vi "GetHSL.vi"(0 "ColorHLS in":refnum<class "ColorHSL.lvclass">, 11 "error in (no error)":errorcluster) -> (4 "ColorHLS out":refnum<class "ColorHSL.lvclass">, 6 "H (°)":dbl, 8 "S (%)":dbl, 10 "L (%)":dbl, 15 "error out":errorcluster)   [LabVIEW 2021, in "Picture2D.lvlib" / "ColorHSL.lvclass"]
uses:
  ColorHSL.lvclass
  ColorHSL.lvclass/ColorHSL.ctl
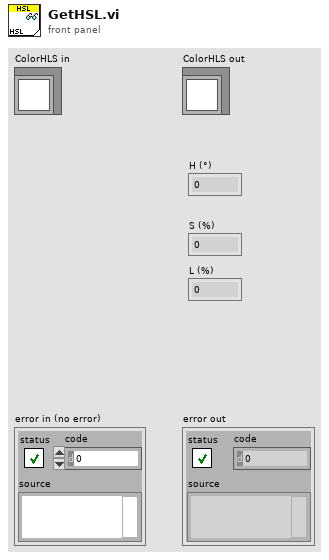
[diagram p1: front panel]
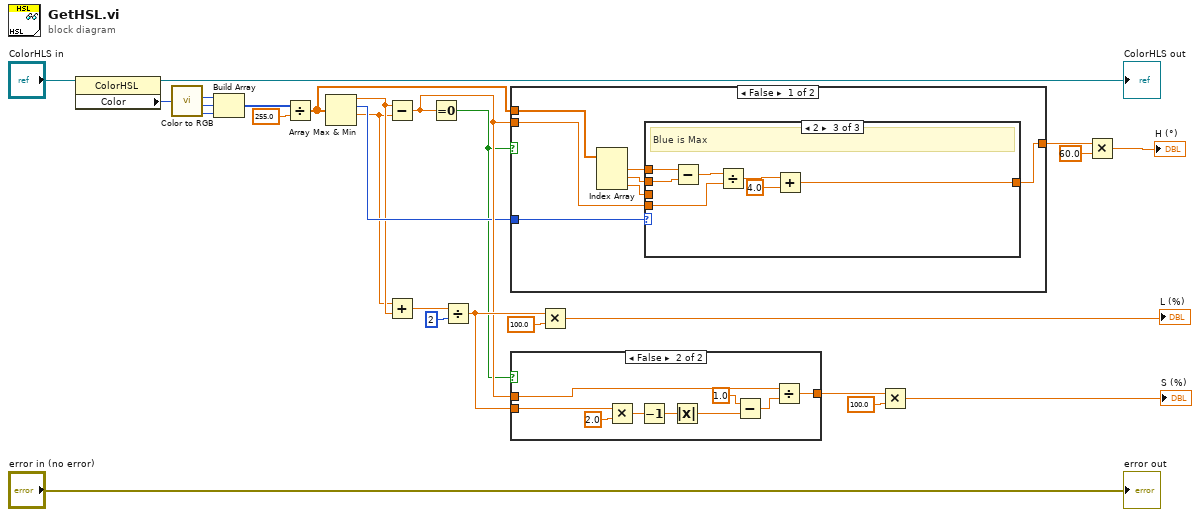
[diagram p0: block diagram]
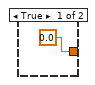
[diagram p2: hidden frame]
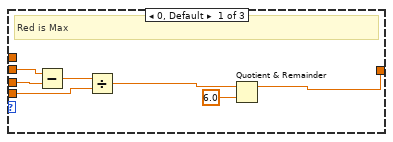
[diagram p3: hidden frame]
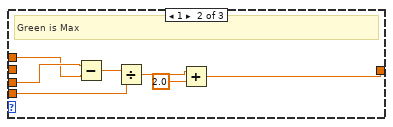
[diagram p4: hidden frame]
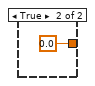
[diagram p5: hidden frame]
diagram:
  n1 = property class="ColorHSL"(reference="ColorHLS in") -> (reference out=→"ColorHLS out":refnum<class "ColorHSL.lvclass">, "Color"=w23:u32)  [unwired: 1 in, 1 out]
  n2 = call <vilib>:"Color to RGB.vi"("Color"=w23) -> ("R"=w11:u8, "G"=w10:u8, "B"=w9:u8)  [unwired: 1 out]
  n3 = Build Array(w11, w10, w9) -> (w20:u8[])
  n4 = Divide(x=w20, y=255.0 ("x")) -> (x/y=w18:dbl[])
  n5 = Array Max & Min(array=w18) -> (max value=w6:dbl, max index (indices)=w7:i32, min value=w5:dbl)  [unwired: 1 out]
  n6 = Subtract(x=w6, y=w5) -> (x-y=w8:dbl)
  n7 = Add(x=w5, y=w6) -> (x+y=w22:dbl)
  n8 = Equal To 0?(x=w8) -> (x = 0?=w4:bool)
  n9 = Divide(x=w22, y=u8 2) -> (x/y=w14:dbl)
  n10 = case shown="False" w4 {
    tunnel: [w32 0.0] -> w17
    tunnel: w7 -> [w33 _]
    tunnel: w18 -> [w31 _]
    tunnel: w8 -> [w27 _]
    frame False {
      n11 = Index Array(array=w31) -> (element #1=w30:dbl, element #2=w29:dbl, element #3=w28:dbl)  [unwired: 3 in]
      n12 = case shown="2" w33 {
        tunnel: w27 -> [w39 w45 w53]
        tunnel: [w34 w41 w51] -> w32
        tunnel: w30 -> [_ w46 w50]
        tunnel: w29 -> [w38 _ w49]
        tunnel: w28 -> [w37 w47 _]
        frame 0, Default {
          # "Red is Max"
          n13 = Subtract(x=w38, y=w37) -> (x-y=w40:dbl)
          n14 = Divide(x=w40, y=w39) -> (x/y=w36:dbl)
          n15 = Quotient & Remainder(x=w36, y=6.0) -> (x-y*floor(x/y)=w34:dbl)  [unwired: 1 out]
        }
        frame 1 {
          # "Green is Max"
          n16 = Subtract(x=w47, y=w46) -> (x-y=w44:dbl)
          n17 = Divide(x=w44, y=w45) -> (x/y=w43:dbl)
          n18 = Add(x=w43, y=2.0) -> (x+y=w41:dbl)
        }
        frame 2 {
          # "Blue is Max"
          n19 = Subtract(x=w50, y=w49) -> (x-y=w54:dbl)
          n20 = Divide(x=w54, y=w53) -> (x/y=w52:dbl)
          n21 = Add(x=w52, y=4.0) -> (x+y=w51:dbl)
        }
      }
    }
    frame True {
    }
  }
  n22 = case shown="False" w4 {
    tunnel: [0.0 ("y") w57] -> w12
    tunnel: w8 -> [_ w65]
    tunnel: w14 -> [_ w64]
    frame True {
    }
    frame False {
      n23 = Multiply(x=w64, y=2.0) -> (x*y=w62:dbl)
      n24 = Decrement(x=w62) -> (x-1=w61:dbl)
      n25 = Absolute Value(x=w61) -> (abs(x)=w60:dbl)
      n26 = Subtract(x=1.0 ("y"), y=w60) -> (x-y=w58:dbl)
      n27 = Divide(x=w65, y=w58) -> (x/y=w57:dbl)
    }
  }
  n28 = Multiply(x=w14, y=100.0) -> (x*y=→"L (%)":dbl)
  n29 = Multiply(x=w12, y=100.0) -> (x*y=→"S (%)":dbl)
  n30 = Multiply(x=w17, y=60.0) -> (x*y=→"H (°)":dbl)
  "error out" <- "error in (no error)"
